vi "rect_lidar_roi.vi"(6 "y_range":i32, 9 "y_center":i32, 10 "x_range":i32, 11 "x_center":i32) -> (2 "y":i32[](array[numeric]), 3 "x":i32[](array[numeric]))   [LabVIEW 2024]
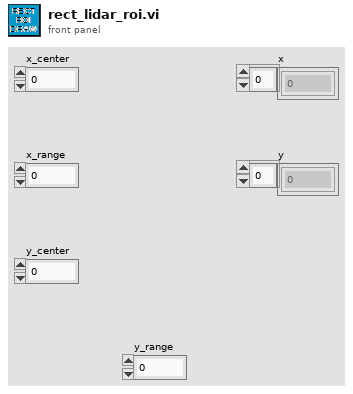
[diagram p1: front panel]
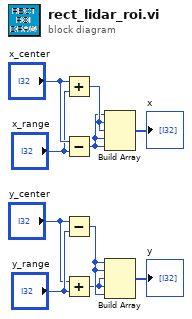
[diagram p0: block diagram]
diagram:
  n1 = Add(x="x_center", y="x_range") -> (x+y=w6:i32)
  n2 = Subtract(x="x_center", y="x_range") -> (x-y=w5:i32)
  n3 = Subtract(x="y_center", y="y_range") -> (x-y=w8:i32)
  n4 = Add(x="y_center", y="y_range") -> (x+y=w7:i32)
  n5 = Build Array(w5, w6, w6, w5, w5) -> (→"x":i32[])
  n6 = Build Array(w8, w8, w7, w7, w8) -> (→"y":i32[])
